vi "Sous_VI_RT_Seaux.vi"(8 "Erreur IN":errorcluster caption="Erreur", 9 "Nombre Sceau IN":i32, 10 "Compteur IN":i32, 11 "Etat IN":T1) -> (0 "Erreur OUT":errorcluster caption="Erreur", 1 "Nombre Sceau OUT":i32, 2 "Compteur OUT":i32, 3 "Etat OUT":T1, 4 "Indicateur de fin de process":bool, 5 "Détection ligne":bool[](array[boolean]))   [LabVIEW 2018]
uses:
  enum_RT_Seaux.ctl
  enum_bras.ctl
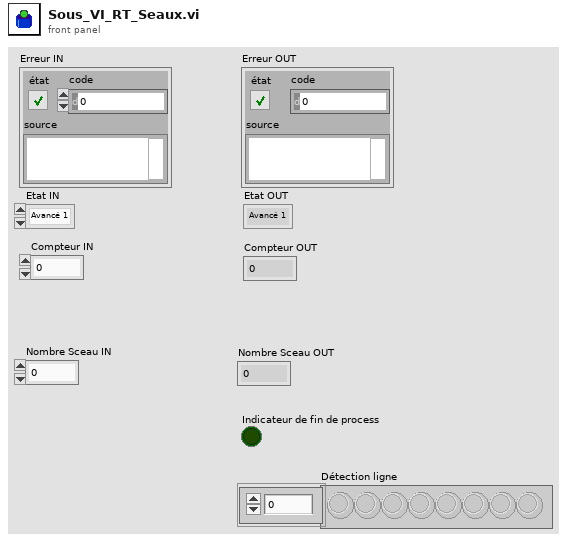
[diagram p1: front panel]
types:
  T1 = typedef "enum_RT_Seaux.ctl" = enum16{"Avancé 1", "Ready to Start", "Stop moteur", "Bras Inactif 1", "Frappe sceau", "Bras Inactif 2", "Avancé 2"}
  T2 = typedef "enum_bras.ctl" = enum16{"Depart Bras", "Clapet Bras", "Inactif Bras", "Seaux Bras"}
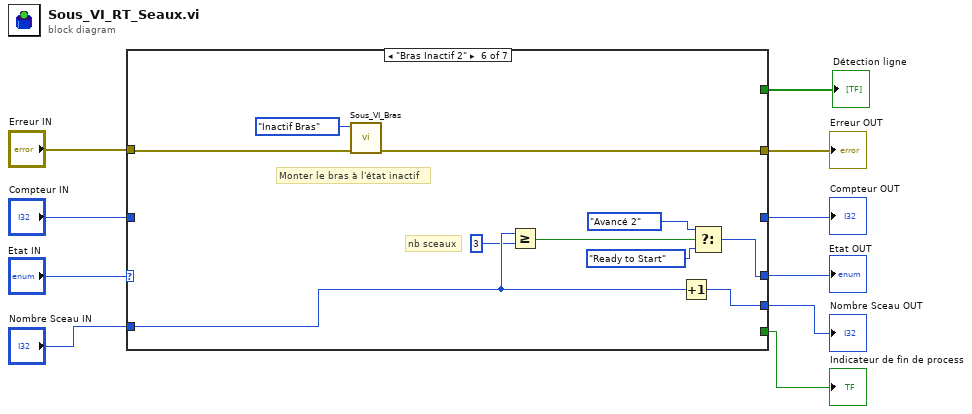
[diagram p0: block diagram]
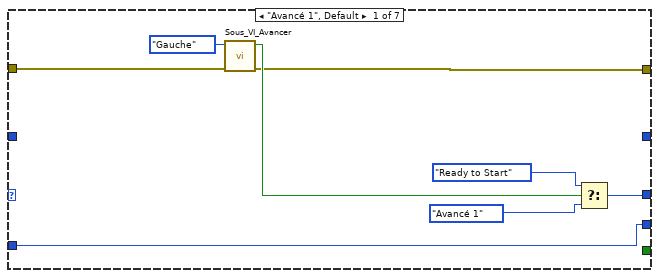
[diagram p2: hidden frame]
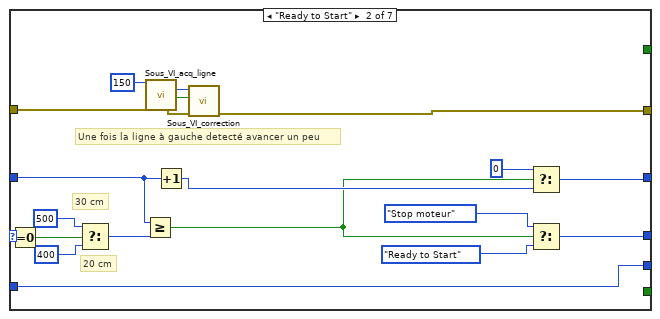
[diagram p3: hidden frame]
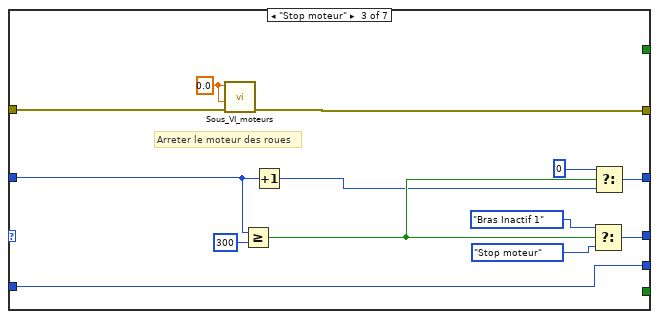
[diagram p4: hidden frame]
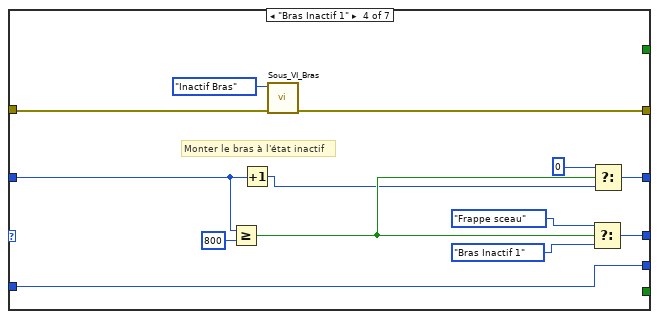
[diagram p5: hidden frame]
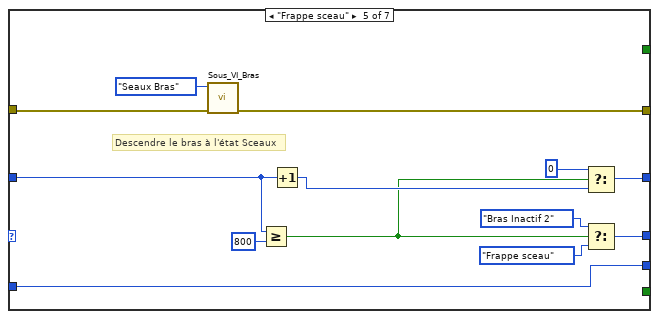
[diagram p6: hidden frame]
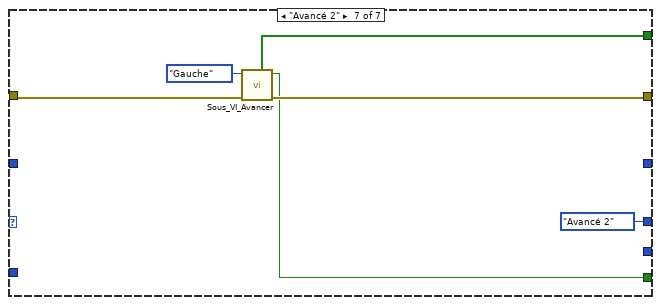
[diagram p7: hidden frame]
diagram:
  n1 = case shown="\"Bras Inactif 2\"" "Etat IN" {
    tunnel: "Erreur IN" -> [w14 w20 w49 w62 w74 w85 w91]
    tunnel: [w15 w24 w48 w61 w75 w84 w90] -> w9
    tunnel: [_ w23 w44 w56 w70 _ _] -> w5
    tunnel: "Compteur IN" -> [_ w21 w47 w58 w72 _ _]
    tunnel: [w12 w22 w46 w59 w71 w78 enum_RT_Seaux."Avancé 2"] -> w7
    tunnel: [w11 w19 w40 w53 w66 w83 _] -> w3
    tunnel: "Nombre Sceau IN" -> [w11 w19 w40 w53 w66 w82 _]
    tunnel: [_ _ _ _ _ _ w89] -> w2
    tunnel: [_ _ _ _ _ _ w88] -> w1
    frame "Avancé 1", Default {
      n2 = call "Sous_VI_Avancer.vi"("error in (no error)"=w14, "Énum"=enum16{"Droite", "Gauche"}."Gauche") -> ("error out"=w15:errorcluster, "Info de fin de Parcours"=w16:bool)  [unwired: 7 in, 1 out]
      n3 = Select(t=enum_RT_Seaux."Ready to Start", s=w16, f=enum_RT_Seaux."Avancé 1") -> (s? t:f=w12:T1)
    }
    frame "Ready to Start" {
      # "20 cm"
      # "30 cm"
      # "Une fois la ligne à gauche detecté avancer un peu"
      n4 = Equal To 0?(x=w19) -> (x = 0?=w30:bool)
      n5 = Select(t=500 ("y"), s=w30, f=400 ("y")) -> (s? t:f=w27:i32)
      n6 = Greater Or Equal?(x=w21, y=w27) -> (x >= y?=w31:bool)
      n7 = call "Sous_VI_acq_ligne.vi"("Seuil"=150, "error in (no error)"=w20) -> ("Décalage"=w37:u32, "G/D ?"=w35:bool, "error out"=w34:errorcluster)  [unwired: 8 in, 3 out]
      n8 = Increment(x=w21) -> (x+1=w32:i32)
      n9 = call "Sous_VI_correction.vi"("error in (no error)"=w34, "G/D ?"=w35, "Décalage"=w37) -> ("error out"=w24:errorcluster)  [unwired: 8 in]
      n10 = Select(t=0, s=w31, f=w32) -> (s? t:f=w23:i32)
      n11 = Select(t=enum_RT_Seaux."Stop moteur", s=w31, f=enum_RT_Seaux."Ready to Start") -> (s? t:f=w22:T1)
    }
    frame "Stop moteur" {
      w50 = 0.0 ("Moteur Gauche")
      # "Arreter le moteur des roues"
      n12 = call "Sous_VI_moteurs.vi"("error in (no error)"=w49, "Moteur Droit"=w50, "Moteur Gauche"=w50) -> ("error out"=w48:errorcluster)  [unwired: 8 in]
      n13 = Greater Or Equal?(x=w47, y=300) -> (x >= y?=w43:bool)
      n14 = Increment(x=w47) -> (x+1=w42:i32)
      n15 = Select(t=enum_RT_Seaux."Bras Inactif 1", s=w43, f=enum_RT_Seaux."Stop moteur") -> (s? t:f=w46:T1)
      n16 = Select(t=0, s=w43, f=w42) -> (s? t:f=w44:i32)
    }
    frame "Bras Inactif 1" {
      # "Monter le bras à l'état inactif"
      n17 = Greater Or Equal?(x=w58, y=800) -> (x >= y?=w55:bool)
      n18 = Increment(x=w58) -> (x+1=w54:i32)
      n19 = call "Sous_VI_Bras.vi"("error in (no error)"=w62, "Enum bras"=enum_bras."Inactif Bras") -> ("error out"=w61:errorcluster)  [unwired: 9 in]
      n20 = Select(t=enum_RT_Seaux."Frappe sceau", s=w55, f=enum_RT_Seaux."Bras Inactif 1") -> (s? t:f=w59:T1)
      n21 = Select(t=0, s=w55, f=w54) -> (s? t:f=w56:i32)
    }
    frame "Frappe sceau" {
      # "Descendre le bras à l'état Sceaux"
      n22 = call "Sous_VI_Bras.vi"("error in (no error)"=w74, "Enum bras"=enum_bras."Seaux Bras") -> ("error out"=w75:errorcluster)  [unwired: 9 in]
      n23 = Greater Or Equal?(x=w72, y=800) -> (x >= y?=w67:bool)
      n24 = Increment(x=w72) -> (x+1=w69:i32)
      n25 = Select(t=0, s=w67, f=w69) -> (s? t:f=w70:i32)
      n26 = Select(t=enum_RT_Seaux."Bras Inactif 2", s=w67, f=enum_RT_Seaux."Frappe sceau") -> (s? t:f=w71:T1)
    }
    frame "Bras Inactif 2" {
      # "nb sceaux"
      # "Monter le bras à l'état inactif"
      n27 = call "Sous_VI_Bras.vi"("error in (no error)"=w85, "Enum bras"=enum_bras."Inactif Bras") -> ("error out"=w84:errorcluster)  [unwired: 9 in]
      n28 = Greater Or Equal?(x=w82, y=3) -> (x >= y?=w77:bool)
      n29 = Increment(x=w82) -> (x+1=w83:i32)
      n30 = Select(t=enum_RT_Seaux."Avancé 2", s=w77, f=enum_RT_Seaux."Ready to Start") -> (s? t:f=w78:T1)
    }
    frame "Avancé 2" {
      n31 = call "Sous_VI_Avancer.vi"("error in (no error)"=w91, "Énum"=enum16{"Droite", "Gauche"}."Gauche") -> ("error out"=w90:errorcluster, "Info de fin de Parcours"=w89:bool, "Détection ligne"=w88:bool[])  [unwired: 7 in]
    }
  }
  "Erreur OUT" <- w9
  "Etat OUT" <- w7
  "Compteur OUT" <- w5
  "Nombre Sceau OUT" <- w3
  "Indicateur de fin de process" <- w2
  "Détection ligne" <- w1
